vi "Example_Loopback_Send.vi"(7 "period":u32, 8 "error in (no error)":errorcluster, 9 "stats in":T1, 10 "tx id":u32 format="%.0x", 11 "channel in":refnum<class "CANsub_Channel.lvclass">) -> (0 "error out":errorcluster, 1 "stats out":T1, 3 "channel out":refnum<class "CANsub_Channel.lvclass">)   [LabVIEW 2021]
doc: "Example: sends frame number sent (4 bytes big-endian) with Write_Frame, stores the send time (High Resolution Relative Seconds) at sent mod 256, schedules the next send one period later."
uses:
  api/CANsub_Channel/CANsub_Channel.lvclass
  Example_Loopback_Stats.ctl
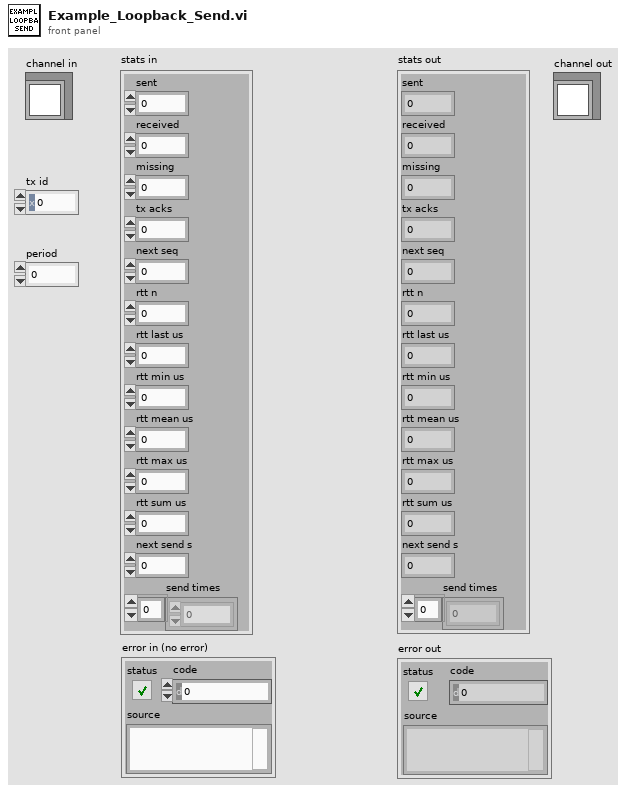
[diagram p1: front panel]
types:
  T1 = typedef "Example_Loopback_Stats.ctl" = cluster{"sent":u32, "received":u32, "missing":u32, "tx acks":u32, "next seq":u32, "rtt n":u32, "rtt last us":dbl, "rtt min us":dbl, "rtt mean us":dbl, "rtt max us":dbl, "rtt sum us":dbl, "next send s":dbl, "send times":dbl[]}
  T2 = enum16{"big-endian, network order", "native, host order", "little-endian"}
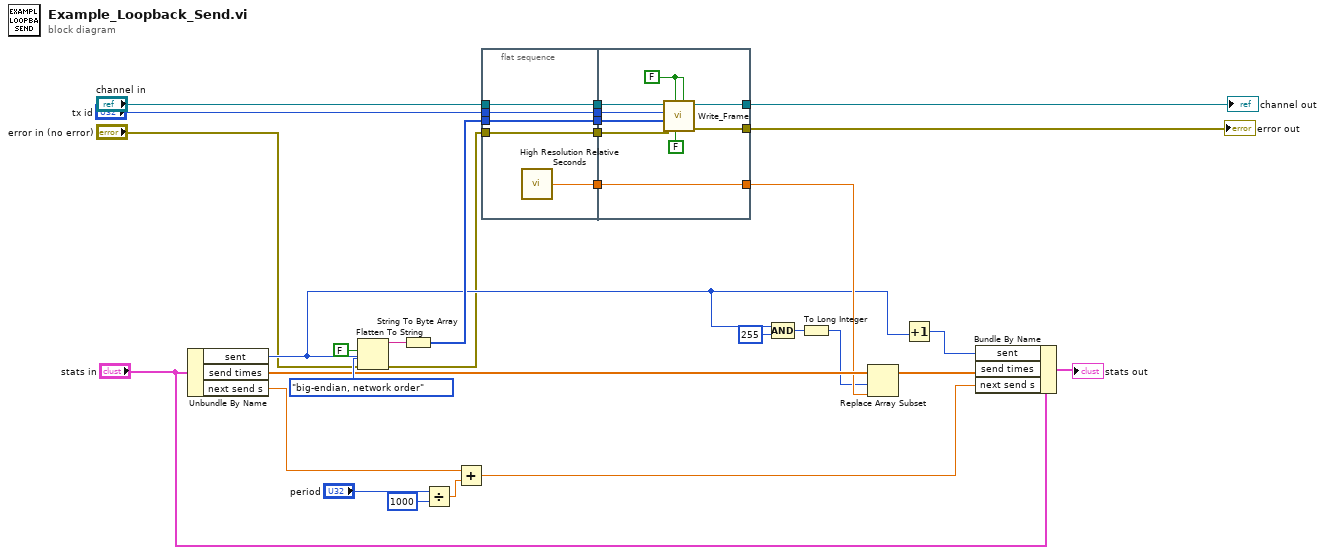
[diagram p0: block diagram]
diagram:
  n1 = Unbundle By Name("stats in") -> ("sent"=w10:u32, "send times"=w16:dbl[], "next send s"=w5:dbl)
  n2 = Flatten To String(anything=w10, prepend array or string size? (T)=FALSE, byte order (0:big-endian, network order)=T2."big-endian, network order", error in (no error)="error in (no error)") -> (data string=w28:string, error out=w2:errorcluster)  [unwired: 1 out]
  n3 = String To Byte Array(string=w28) -> (unsigned byte array=w21:u8[])
  n4 = Divide(x="period", y=u32 1000) -> (x/y=w6:dbl)
  n5 = Add(x=w5, y=w6) -> (x+y=w4:dbl)
  n6 = flat-sequence {
    tunnel: [w35] -> w27
    tunnel: [w34] -> w25
    tunnel: "channel in" -> [w34]
    tunnel: [w33] -> w22
    tunnel: w21 -> [w33]
    tunnel: [w32] -> w20
    tunnel: "tx id" -> [w32]
    tunnel: [w31] -> w18
    tunnel: w2 -> [w31]
    tunnel: w27 -> [w36]
    tunnel: w25 -> [w44]
    tunnel: [w43] -> w23
    tunnel: w22 -> [w42]
    tunnel: w20 -> [w41]
    tunnel: w18 -> [w40]
    tunnel: [w37] -> w17
    tunnel: [w36] -> w15
    frame #0 {
      n7 = call <vilib>:"High Resolution Relative Seconds.vi"() -> ("relative seconds"=w35:dbl)
    }
    frame #1 {
      w39 = FALSE ("ide")
      n8 = call-dynamic "Write_Frame.vi"("fdf"=w39, "brs"=FALSE, "ide"=w39, "error in (no error)"=w40, "data"=w42, "id"=w41, "channel in"=w44) -> ("error out"=w37:errorcluster, "channel out"=w43:refnum<class "CANsub_Channel.lvclass">)  [unwired: 3 in]
    }
  }
  n9 = Compound Arithmetic op=AND(w10, u32 255 ("value")) -> (w13:u32)
  n10 = To Long Integer(number=w13) -> (32bit integer=w11:i32)
  n11 = Replace Array Subset(array=w16, new element=w15, index=w11) -> (w12:dbl[])
  n12 = Increment(x=w10) -> (x+1=w9:u32)
  n13 = Bundle By Name(cluster="stats in", "sent"=w9, "send times"=w12, "next send s"=w4) -> (→"stats out":T1)
  "channel out" <- w23
  "error out" <- w17
